vi "Test U8 Backpressure.vi"() -> ()   [LabVIEW 2021]
uses:
  ChannelCommon/typedef/Direction.ctl
  ChannelCommon/typedef/TimeStamps.ctl
  CIF_Iceoryx_PCAP_Universal.lvclass
  ChannelCommon/typedef/New FIFO Instance Configuration.ctl
  Iceorxy Utilities/Typedef/PCAP Config.ctl
  ChannelCommon/typedef/New FIFO Config.ctl
  ChannelCommon/typedef/FIFO Flags.ctl
  Iceorxy Utilities/Typedef/PCAP Linktype.ctl
  ChannelCommon/ChannelCommon.lvlib
  Iceorxy Utilities/Iceoryx Channel Utilities.lvlib
panel:
  out "status":string
  out "pass":bool
  out "error out":errorcluster
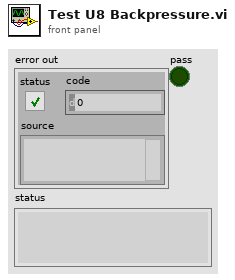
[diagram p1: front panel]
types:
  T1 = typedef "ChannelCommon.lvlib/Direction.ctl" = enum8{"Publisher", "Subscriber"}
  T2 = typedef "Iceoryx Channel Utilities.lvlib/PCAP Config.ctl" = cluster{"New FIFO Config":T3, "Linktype":T5, "Linktype Override":u32, "Type Name Override":string}
  T3 = typedef "ChannelCommon.lvlib/New FIFO Config.ctl" = cluster{"Max Bytes/Msg":u64, "Max Msg/FIFO":u64, "FIFO Flags":T4, "Best Effort Subscribers":u32, "Backpressure Subscribers":u32}
  T4 = typedef "ChannelCommon.lvlib/FIFO Flags.ctl" = cluster{"Backpressure":bool, "Extended Config":bool}
  T5 = typedef "Iceoryx Channel Utilities.lvlib/PCAP Linktype.ctl" = u32
  T6 = typedef "ChannelCommon.lvlib/New FIFO Instance Configuration.ctl" = cluster{"Backpressure":bool, "Bytes/Message Override":u32, "Messages/FIFO Override":u32, "Custom Data":u8[]}
  T7 = typedef "ChannelCommon.lvlib/TimeStamps.ctl" = cluster{"ClockID":u8, "T0":i64, "T_Out":i64}
  T8 = typedef "ChannelCommon.lvlib/New FIFO Instance Response.ctl" = cluster{"Publisher":string, "Custom Data":u8[]}
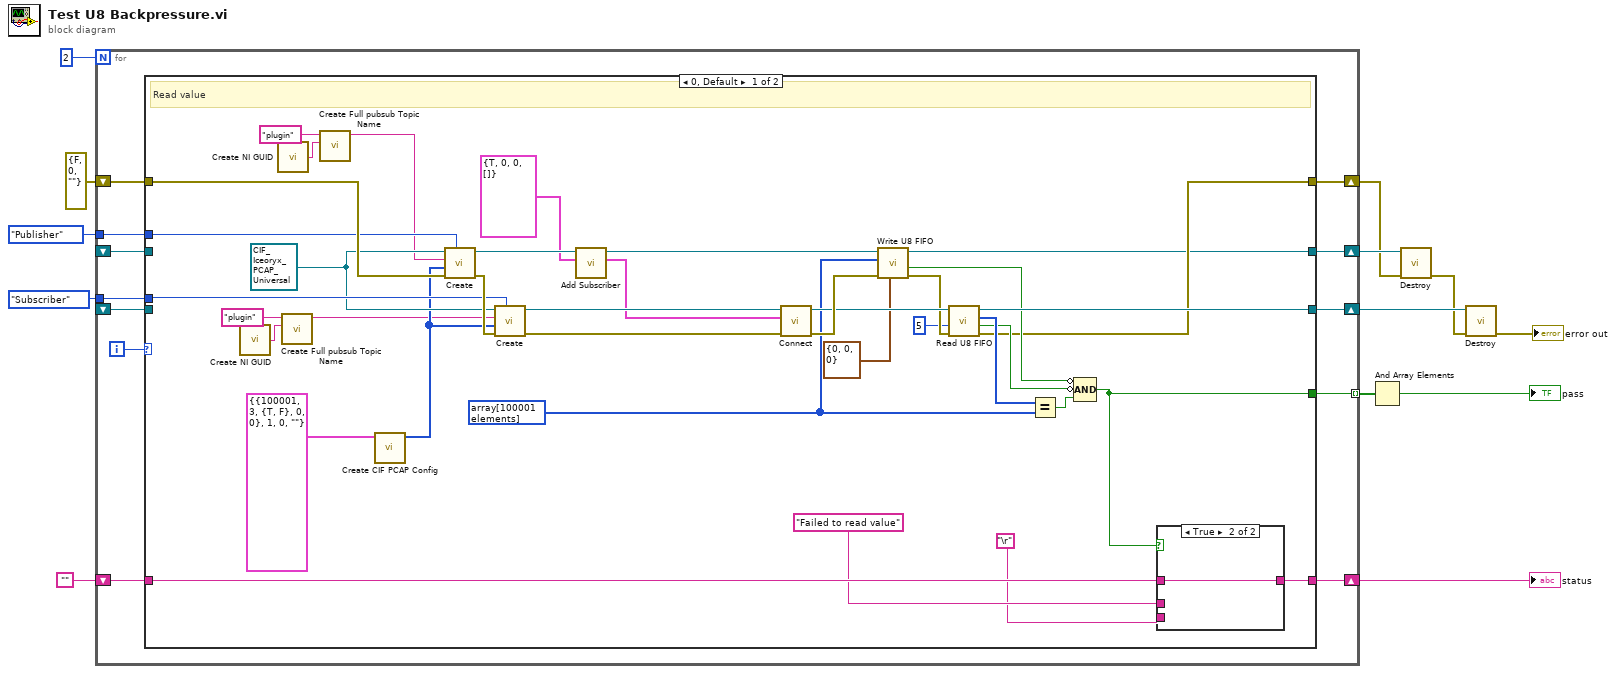
[diagram p0: block diagram]
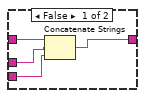
[diagram p2: hidden frame]
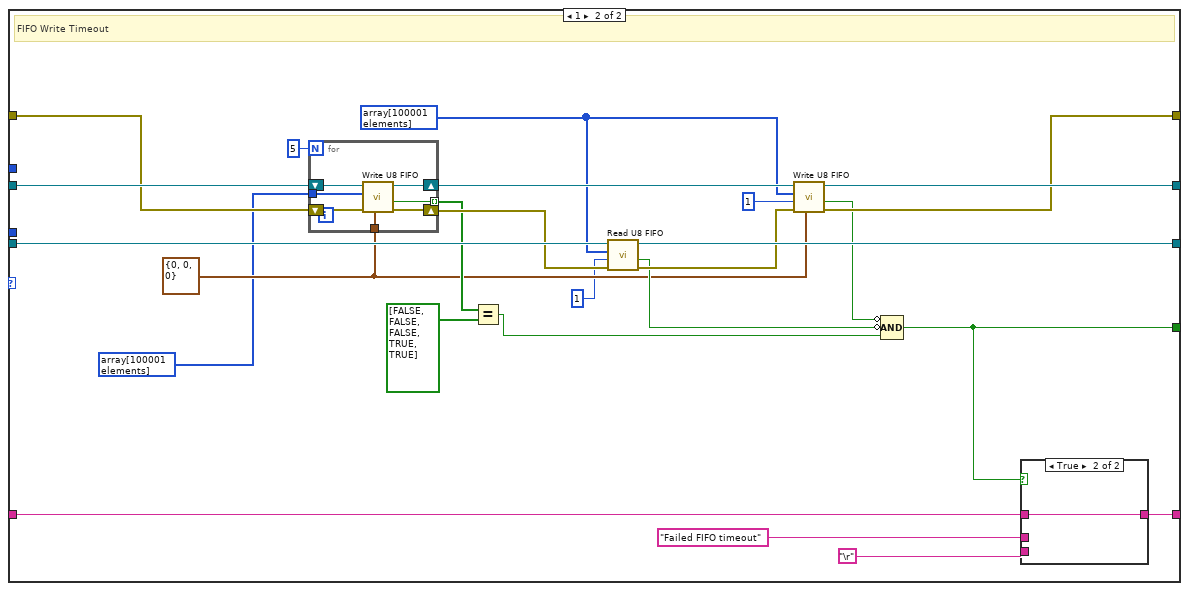
[diagram p3: hidden frame]
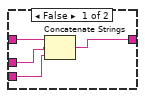
[diagram p4: hidden frame]
diagram:
  n1 = for {
    N: 2 -> [_]
    tunnel: [w25] -> w13 mode=indexing
    shift-right: [w23] -> w4
    shift-left: errorcluster {"status"=FALSE, "code"=0, "source"=""} ("error out") -> [w24]
    shift-right: [w20] -> w9
    shift-left: "" -> [w21]
    tunnel: Direction."Subscriber" ("Direction") -> [w19]
    tunnel: Direction."Publisher" ("Direction") -> [w18]
    shift-right: [w17] -> w3
    shift-left: _ -> [w15]
    shift-right: [w16] -> w5
    shift-left: _ -> [w14]
    i -> [w22]
    n2 = case shown="0, Default" w22 {
      tunnel: [w57 w73] -> w25
      tunnel: w24 -> [w55 w87]
      tunnel: [w39 w79] -> w23
      tunnel: w21 -> [w62 w92]
      tunnel: [w61 w91] -> w20
      tunnel: w19 -> [w54 _]
      tunnel: w18 -> [w53 _]
      tunnel: [w48 w84] -> w17
      tunnel: [w38 w82] -> w16
      tunnel: w14 -> [_ w88]
      tunnel: w15 -> [_ w85]
      frame 0, Default {
        w43 = refnum<class "CIF_Iceoryx_PCAP_Universal.lvclass"> refnum ("CIF_CIPC_Fifo_U8.lvclass")
        w40 = u8[] array[100001 elements] ("U8 Data")
        # "Read value"
        n3 = call <vilib>:"Create NI GUID.vi"() -> ("NI GUID"=w27:string)
        n4 = call <vilib>:"Create NI GUID.vi"() -> ("NI GUID"=w31:string)
        n5 = call "Create Full pubsub Topic Name.vi"("Topic"=w27, "Plugin name"="plugin") -> ("Full Topic"=w26:string)  [unwired: 8 in, 1 out]
        n6 = call "Create Full pubsub Topic Name.vi"("Topic"=w31, "Plugin name"="plugin") -> ("Full Topic"=w29:string)  [unwired: 8 in, 1 out]
        n7 = call "Create CIF PCAP Config.vi"("PCAP FIFO Config"=T2 {"New FIFO Config"={"Max Bytes/Msg"=100001, "Max Msg/FIFO"=3, "FIFO Flags"={"Backpressure"=TRUE, "Extended Config"=FALSE}, "Best Effort Subscribers"=0, "Backpressure Subscribers"=0}, "Linktype"=1, "Linktype Override"=0, "Type Name Override"=""}) -> ("Flattened PCAP FIFO Config"=w32:u8[])  [unwired: 10 in]
        n8 = call-dynamic "Create.vi"("Direction"=w53, "error in (no error)"=w55, "Custom Config Data"=w32, "Name"=w29, "CIFFIFO in"=w43) -> ("error out"=w56:errorcluster, "CIFFIFO out"=w37:refnum<class "CIF_Iceoryx_PCAP_Universal.lvclass">)  [unwired: 5 in]
        n9 = call-dynamic "Create.vi"("Direction"=w54, "error in (no error)"=w56, "Custom Config Data"=w32, "Name"=w26, "CIFFIFO in"=w43) -> ("error out"=w52:errorcluster, "CIFFIFO out"=w51:refnum<class "CIF_Iceoryx_PCAP_Universal.lvclass">)  [unwired: 5 in]
        n10 = call-dynamic "Add Subscriber.vi"("New FIFO Instance Config"=T6 {"Backpressure"=TRUE, "Bytes/Message Override"=0, "Messages/FIFO Override"=0, "Custom Data"=[]}, "CIF_CIPC_Chn in"=w37) -> ("New FIFO Instance"=w35:T8, "CIF_CIPC_Chn out"=w36:refnum<class "CIF_Iceoryx_PCAP_Universal.lvclass">)  [unwired: 7 in, 1 out]
        n11 = call-dynamic "Connect.vi"("error in (no error)"=w52, "Connection"=w35, "CIF_Iceoryx_PCAP"=w51) -> ("error out"=w50:errorcluster, "CIF_Iceoryx_PCAP"=w49:refnum<class "CIF_Iceoryx_PCAP_Universal.lvclass">)  [unwired: 7 in]
        n12 = call-dynamic "Write U8 FIFO.vi"("FIFO Timestamps"=T7 {"ClockID"=0, "T0"=0, "T_Out"=0}, "error in (no error)"=w50, "Data in"=w40, "CIFFIFO in"=w36) -> ("error out"=w47:errorcluster, "timed out?"=w46:bool, "CIFFIFO out"=w38:refnum<class "CIF_Iceoryx_PCAP_Universal.lvclass">)  [unwired: 4 in, 1 out]
        n13 = call-dynamic "Read U8 FIFO.vi"("error in (no error)"=w47, "Timeout (ms)"=5, "CIFFIFO in"=w49) -> ("error out"=w39:errorcluster, "timed out?"=w44:bool, "Data out"=w45:u8[], "CIFFIFO out"=w48:refnum<class "CIF_Iceoryx_PCAP_Universal.lvclass">)  [unwired: 4 in, 1 out]
        n14 = Equal?(x=w45, y=w40) -> (x = y?=w58:bool)
        n15 = Compound Arithmetic op=AND(invert w46, invert w44, w58) -> (w57:bool)
        n16 = case shown="True" w57 {
          tunnel: w62 -> [w66 w67]
          tunnel: [w63 w67] -> w61
          tunnel: "Failed to read value" -> [w65 _]
          tunnel: "\r" -> [w64 _]
          frame False {
            n17 = Concatenate Strings(w66, w65, w64) -> (w63:string)
          }
          frame True {
          }
        }
      }
      frame 1 {
        w70 = u8[] array[100001 elements] ("U8 Data")
        w72 = T7 {"ClockID"=0, "T0"=0, "T_Out"=0} ("FIFO Timestamps")
        # "FIFO Write Timeout"
        n18 = for {
          N: 5 -> [_]
          tunnel: u8[] array[100001 elements] ("U8 Data") -> [w97]
          tunnel: w72 -> [w96]
          shift-right: [w95] -> w83
          shift-left: w88 -> [w99]
          tunnel: [w94] -> w78 mode=indexing
          shift-right: [w93] -> w81
          shift-left: w87 -> [w98]
          n19 = call-dynamic "Write U8 FIFO.vi"("FIFO Timestamps"=w96, "error in (no error)"=w98, "Data in"=w97, "CIFFIFO in"=w99) -> ("error out"=w93:errorcluster, "timed out?"=w94:bool, "CIFFIFO out"=w95:refnum<class "CIF_Iceoryx_PCAP_Universal.lvclass">)  [unwired: 4 in, 1 out]
        }
        n20 = Equal?(x=w78, y=bool[] [FALSE, FALSE, FALSE, TRUE, TRUE]) -> (x = y?=w74:bool)
        n21 = call-dynamic "Read U8 FIFO.vi"("error in (no error)"=w81, "Timeout (ms)"=1, "Data in"=w70, "CIFFIFO in"=w85) -> ("error out"=w80:errorcluster, "timed out?"=w76:bool, "CIFFIFO out"=w84:refnum<class "CIF_Iceoryx_PCAP_Universal.lvclass">)  [unwired: 3 in, 2 out]
        n22 = call-dynamic "Write U8 FIFO.vi"("FIFO Timestamps"=w72, "error in (no error)"=w80, "Timeout (ms)"=1, "Data in"=w70, "CIFFIFO in"=w83) -> ("error out"=w79:errorcluster, "timed out?"=w75:bool, "CIFFIFO out"=w82:refnum<class "CIF_Iceoryx_PCAP_Universal.lvclass">)  [unwired: 3 in, 1 out]
        n23 = Compound Arithmetic op=AND(invert w75, invert w76, w74) -> (w73:bool)
        n24 = case shown="True" w73 {
          tunnel: w92 -> [w103 w104]
          tunnel: [w100 w104] -> w91
          tunnel: "Failed FIFO timeout" -> [w102 _]
          tunnel: "\r" -> [w101 _]
          frame False {
            n25 = Concatenate Strings(w103, w102, w101) -> (w100:string)
          }
          frame True {
          }
        }
      }
    }
  }
  "status" <- w9
  n26 = And Array Elements(Boolean array=w13) -> (logical AND=→"pass":bool)
  n27 = call-dynamic "Destroy.vi"("error in (no error)"=w4, "Icoryx_PCAP in"=w5) -> ("error out"=w2:errorcluster)  [unwired: 8 in, 1 out]
  n28 = call-dynamic "Destroy.vi"("error in (no error)"=w2, "Icoryx_PCAP in"=w3) -> ("error out"=→"error out":errorcluster)  [unwired: 8 in, 1 out]
